vi "MongoDB.RenameCollection.vi"(8 "error in (no error)":errorcluster, 9 "newCollectionName":string, 10 "oldCollectionName":string, 11 "MongoDB.Database in":refnum<class "MongoDB.Database.lvclass">) -> (0 "error out":errorcluster, 3 "MongoDB.Database out":refnum<class "MongoDB.Database.lvclass">)   [LabVIEW 2014, in "MongoDB.Database.lvclass"]
uses:
  MongoDB.Database.lvclass
  MongoDB.Database.lvclass/MongoDB.Database.ctl
  C:/Users/Richard/Documents/GitHub/mongo-labview-driver/CSharp/bin/MongoDB.Driver.Legacy.dll
  CSharp/bin/MongoDB.Driver.Legacy.dll
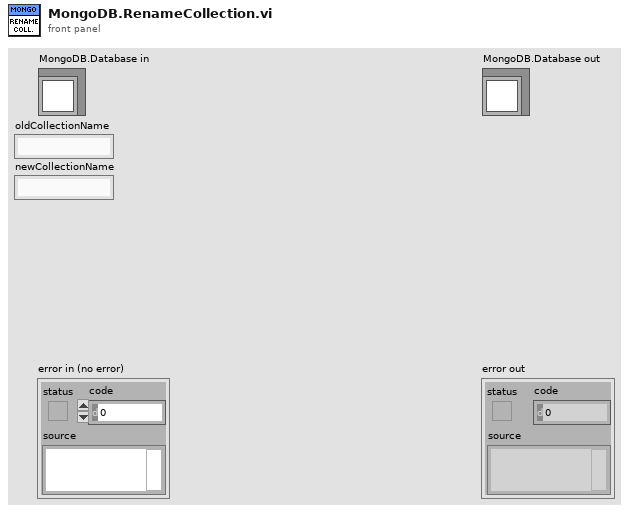
[diagram p1: front panel]
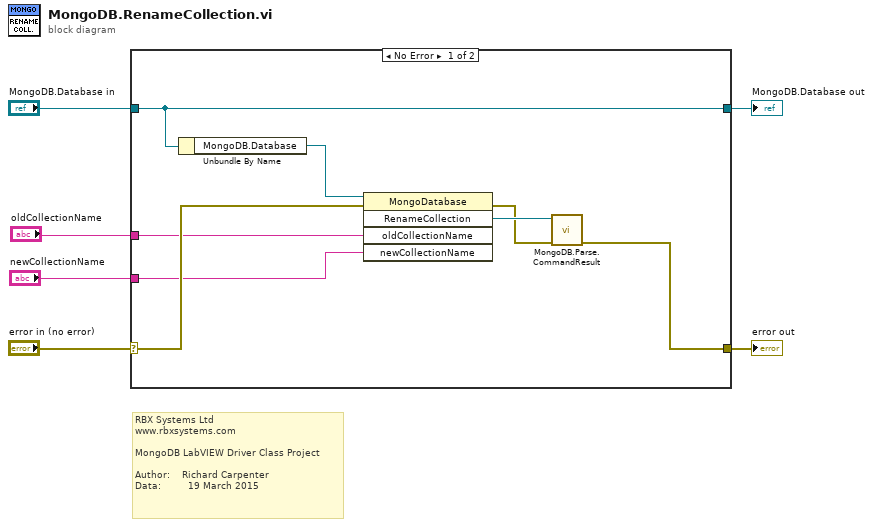
[diagram p0: block diagram]
diagram:
  # "RBX Systems Ltd\nwww.rbxsystems.com\n\nMongoDB LabVIEW Driver Class Project\n\nAuthor:    Richard Carpenter\nData:         19 March 2015"
  n1 = case shown="No Error" "error in (no error)" {
    selector: "error in (no error)" -> [w12 w16]
    tunnel: [w7 w16] -> w5
    tunnel: [w14 w15] -> w3
    tunnel: "MongoDB.Database in" -> [w14 w15]
    tunnel: "oldCollectionName" -> [w11 _]
    tunnel: "newCollectionName" -> [w10 _]
    frame No Error {
      n2 = Unbundle By Name(w14) -> ("MongoDB.Database"=w13:refnum<k24>)
      n3 = invoke class="MongoDatabase" method="RenameCollection"(reference=w13, error in=w12, "oldCollectionName"=w11, "newCollectionName"=w10) -> (error out=w8:errorcluster, "RenameCollection"=w9:refnum<k24>)  [unwired: 1 in, 3 out]
      n4 = call "MongoDB.Parse.CommandResult.vi"("error in (no error)"=w8, "MongoDB.Command.Result"=w9) -> ("error out"=w7:errorcluster)  [unwired: 9 in]
    }
    frame Error {
    }
  }
  "error out" <- w5
  "MongoDB.Database out" <- w3
